vi "C.vi"(11 "error in":errorcluster) -> (15 "error out":errorcluster)   [LabVIEW 2026]
doc: "Repro caller outside the class: calls Cls.lvclass:Touch.vi on a class constant."
uses:
  Cls/Cls.lvclass
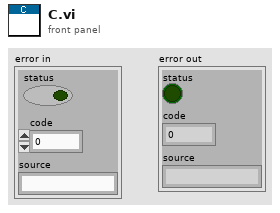
[diagram p1: front panel]
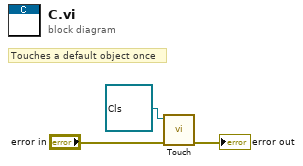
[diagram p0: block diagram]
diagram:
  # "Touches a default object once"
  n1 = call "Touch.vi"("error in"="error in", "Cls in"=refnum<class "Cls.lvclass"> refnum ("Seed1")) -> ("error out"=→"error out":errorcluster)  [unwired: 8 in, 1 out]
